vi "MQTT Data - Encode Varint.vi"(7 "Value":u32) -> (8 "encoded value":u8[](array[numeric]))   [LabVIEW 2019, in "KoRE-MQTT.lvlib"]
doc: "Copyright (c) 2025 KoRElibs.com\nSPDX-License-Identifier: EUPL-1.2\n\nThis VI is licensed under the European Union Public License (EUPL) Version 1.2. You may use this VI unmodified in proprietary works. If you distribute a modified version of this file, the modified file must be released under the EUPL-1.2. Full license: https://joinup.ec.europa.eu/asset/eupl/eupl/1.2/"
uses:
  KoRE-MQTT.lvlib
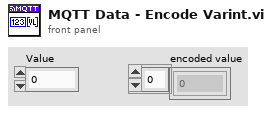
[diagram p1: front panel]
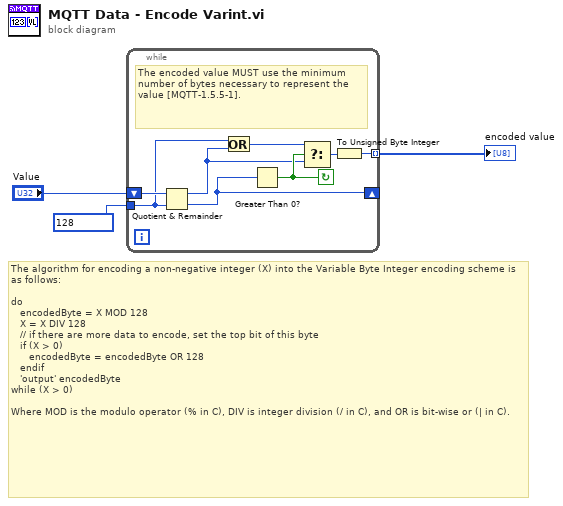
[diagram p0: block diagram]
diagram:
  # "The algorithm for encoding a non-negative integer (X) into the Variable Byte Integer encoding scheme is as follows:\n\ndo\n   encodedByte = X MOD 128\n   X = X DIV 128\n   // if there are more data to encode, set the top bit of this byte\n   if (X > 0)\n      encodedByte = encodedByte OR 128\n   endif\n   'output' encodedByte\nwhile (X > 0)\n\nWhere MOD is the modulo operator (% in C), DIV is integer division (/ in C), and OR is bit-wise or (| in C)."
  n1 = while {
    shift-right: [w7] -> _
    shift-left: "Value" -> [w11]
    tunnel: [w4] -> w1 mode=indexing
    tunnel: u32 128 ("y") -> [w6]
    stop <- w10 continue-if-true
    # "The encoded value MUST use the minimum number of bytes necessary to represent the value [MQTT-1.5.5-1]."
    n2 = Quotient & Remainder(x=w11, y=w6) -> (x-y*floor(x/y)=w5:u32, floor(x/y)=w7:u32)
    n3 = Or(x=w6, y=w5) -> (x .or. y?=w8:u32)
    n4 = Greater Than 0?(x=w7) -> (x > 0?=w10:bool)
    n5 = Select(t=w8, s=w10, f=w5) -> (s? t:f=w9:u32)
    n6 = To Unsigned Byte Integer(number=w9) -> (unsigned 8bit integer=w4:u8)
  }
  "encoded value" <- w1
